vi "control-other-input.vi"(0 "Standard Input":string, 11 "error in":errorcluster) -> (15 "error out":errorcluster)   [LabVIEW 2024]
doc: "Static analysis fixture. Do not run."
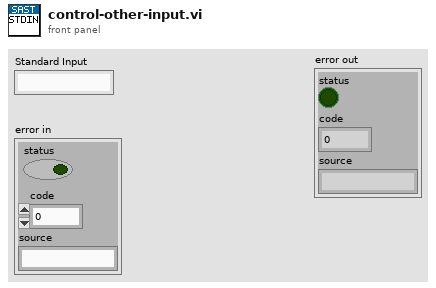
[diagram p1: front panel]
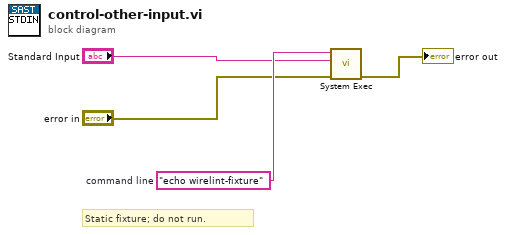
[diagram p0: block diagram]
diagram:
  w3 = "echo wirelint-fixture"  # command line
  # "Static fixture; do not run."
  n1 = call <vilib>:"System Exec.vi"("error in (no error)"="error in", "standard input"="Standard Input", "command line"=w3) -> ("error out"=→"error out":errorcluster)  [unwired: 5 in, 3 out]
